vi "MRC SmartIO API Changes.vi"   [LabVIEW 2023]
uses:
  <vilib>/MRC/MrcLib.lvlib
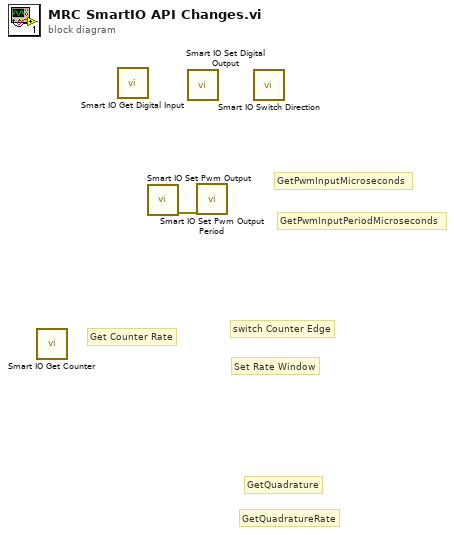
[diagram p0: block diagram]
diagram:
  # "GetQuadratureRate"
  # "GetQuadrature"
  # "Get Counter Rate"
  # "GetPwmInputPeriodMicroseconds"
  # "GetPwmInputMicroseconds"
  # "Set Rate Window"
  # "switch Counter Edge"
  n1 = call <vilib>:"Smart IO Get Counter.vi"() -> ()  [unwired: 10 in, 2 out]
  n2 = call <vilib>:"Smart IO Get Digital Input.vi"() -> ()  [unwired: 10 in, 2 out]
  n3 = call <vilib>:"Smart IO Set Pwm Output.vi"() -> ("error out"=w1:errorcluster)  [unwired: 11 in]
  n4 = call <vilib>:"Smart IO Set Digital Output.vi"() -> ()  [unwired: 11 in, 1 out]
  n5 = call <vilib>:"Smart IO Set Pwm Output Period.vi"("error in (no error)"=w1) -> ()  [unwired: 10 in, 1 out]
  n6 = call <vilib>:"Smart IO Switch Direction.vi"() -> ()  [unwired: 11 in, 1 out]
